vi "ZM-CP-FL-createFolder.vi"(8 "error in (no error)":errorcluster, 11 "ZM-CP-communication_protocol in":refnum<class "ZM-CP-communication_protocol.lvclass">) -> (0 "error out":errorcluster, 3 "ZM-CP-communication_protocol out":refnum<class "ZM-CP-communication_protocol.lvclass">)   [LabVIEW 2020, in "ZM-CP-FL-file_logger.lvlib" / "ZM-CP-FL-file_logger.lvclass"]
doc: "Hook of the file logger, called by its ZM-CP-init override after Call Parent: creates outputFolder if it is missing. An existing folder (code 10) is not an error; every other error passes. The class terminals are typed as the parent so the hook fits the override's dynamic wire."
uses:
  ZM-CP-FL-file_logger.lvclass
  ZM-CP-communication_protocol/ZM-CP-communication_protocol/ZM-CP-communication_protocol.lvclass
  ZM-CP-FL-file_logger.lvclass/ZM-CP-FL-file_logger.ctl
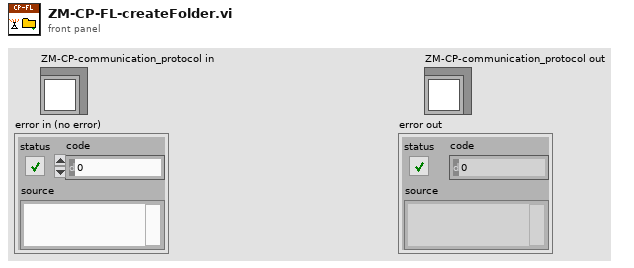
[diagram p1: front panel]
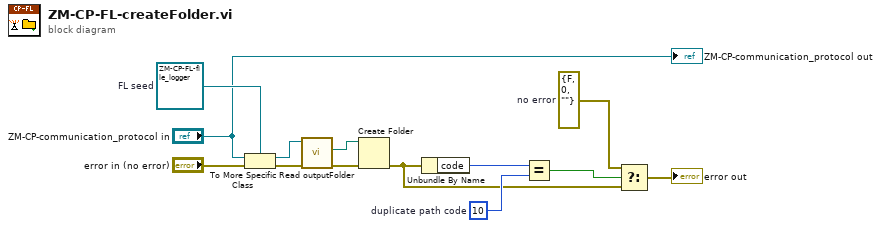
[diagram p0: block diagram]
diagram:
  w5 = errorcluster {"status"=FALSE, "code"=0, "source"=""}  # no error
  w6 = 10  # duplicate path code
  w12 = refnum<class "ZM-CP-FL-file_logger.lvclass"> refnum  # FL seed
  n1 = To More Specific Class(target class=w12, reference="ZM-CP-communication_protocol in", error in="error in (no error)") -> (specific class reference=w10:refnum<class "ZM-CP-FL-file_logger.lvclass">, error out=w11:errorcluster)
  n2 = call "Read outputFolder.vi"("error in (no error)"=w11, "ZM-CP-FL-file_logger in"=w10) -> ("error out"=w8:errorcluster, "outputFolder"=w9:path)  [unwired: 7 in, 1 out]
  n3 = Create Folder(path (use dialog)=w9, error in=w8) -> (error out=w3:errorcluster)  [unwired: 1 in, 2 out]
  n4 = Unbundle By Name(w3) -> ("code"=w7:i32)
  n5 = Equal?(x=w7, y=w6) -> (x = y?=w4:bool)
  n6 = Select(t=w5, s=w4, f=w3) -> (s? t:f=→"error out":errorcluster)
  "ZM-CP-communication_protocol out" <- "ZM-CP-communication_protocol in"
